vi "Sim_VTU_Plant.vi"(8 "error in (no error)":errorcluster={"status"=FALSE, "code"=0, "source"="\"\""}, 9 "displacement_sp":dbl=2.0, 10 "flow_sp":dbl=40.0, 11 "pressure_sp":dbl=100.0) -> (0 "error out":errorcluster={"status"=FALSE, "code"=0, "source"="\"\""}, 1 "act_power_kW":dbl, 2 "act_flow":dbl, 3 "act_pressure":dbl)   [LabVIEW 2026]
doc: "INTENT: Deterministic first-order dynamic plant response for VTU hydraulic hitch and servo. Computes actuator pressure, flow, displacement and hydraulic power."
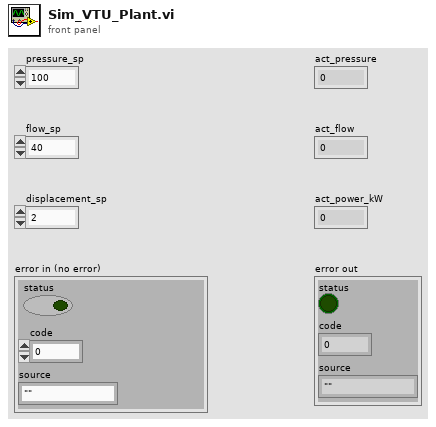
[diagram p1: front panel]
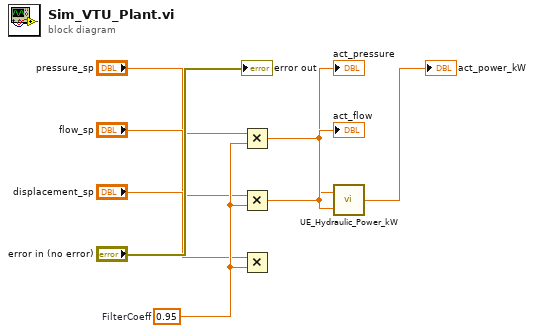
[diagram p0: block diagram]
diagram:
  w5 = 0.95  # FilterCoeff
  n1 = Multiply(x="pressure_sp", y=w5) -> (x*y=w6:dbl)
  "act_pressure" <- w6
  n2 = Multiply(x="flow_sp", y=w5) -> (x*y=w7:dbl)
  "act_flow" <- w7
  n3 = Multiply(x="displacement_sp", y=w5) -> ()  [unwired: 1 out]
  n4 = call "UE_Hydraulic_Power_kW.vi"("flow_lpm"=w7, "pressure_bar"=w6) -> ("hydraulic_kw"=→"act_power_kW":dbl)
  "error out" <- "error in (no error)"
